vi "[ce] CalcExpress Light.vi"(5 "directives":T1={"enaNamedConst"=TRUE}, 7 "VC Handle":T5=-1, 8 "error in":errorcluster, 9 "params":T3={"autoVar"=TRUE, "enCpx"=TRUE}, 10 "repeat (1)":i32=1, 11 "expression":string) -> (0 "error out":errorcluster, 1 "value type":T4=enum."DBL Number", 3 "numeric value":dbl)   [LabVIEW 2021]
doc: "This VI evaluates CalcExpress expressions and sequential scripts. To process non-sequential scripts that contain loops and conditional branching, use <b>CSE VIs</b>. Refer to the VI help for more details.\n\n<b>VC Handle</b> specifies the handle of a variable context. CalcExpress accesses variables using this handle. Pass a valid handle to this terminal if the expression uses variables; otherwise, you can leave this input unwired.\n\n<b>expression</b> specifies the CalcExpress expression or sequential script to be executed.\n\n<b>repeat</b> control specifies the number of times an expression is evaluated. The default value is 1.\n\n<b>params</b> cluster specifies optional parameters influencing evaluation:\n <b>autoVar</b> : if it is TRUE (default) and a non-existent variable appears as the left-hand operand in the assignment operator, CalcExpress implicitly creates the variable. If it is FALSE, all variables in the expression must be explicitly created either before or during evaluation.\n <b>enCpx</b> : enables (TRUE, default) or disables (FALSE) the ability to perform operations on operands of data types other than <b>DBL Number</b>.\n\n<b>numeric value</b> returns the numeric value (<b>DBL Number</b>) of the expression.\n\n<b>value type</b> indicates the data type of the expression value.\n\n::: CalcExpress Toolkit :::\nCopyright (c) 2000-2026 Konstantin Shifershteyn. All rights reserved."
uses:
  cetypes.llb/VarMan Variable Context Handle.ctl
  cetypes.llb/CalcExpress Data Type.ctl
  cetypes.llb/CalcExpress Execution Options.ctl
  cetypes.llb/CalcExpress Instance RefNum.ctl
  cetypes.llb/CalcExpress Parsing Directives.ctl
  cersrc/celveng32.dll
panel:
  in  "CE InstanceRef Templ.":T2
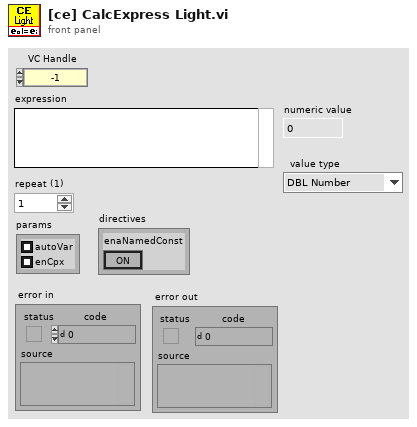
[diagram p1: front panel]
types:
  T1 = typedef "CalcExpress Parsing Directives.ctl" = cluster{"enaNamedConst":bool}
  T2 = typedef "CalcExpress Instance RefNum.ctl" = refnum<k1>
  T3 = typedef "CalcExpress Execution Options.ctl" = cluster{"autoVar":bool, "enCpx":bool}
  T4 = typedef "CalcExpress Data Type.ctl" = enum32{"String", "DBL Number", "identifier", "1D Array of DBL", "2D Array of DBL", "CDB Number", "1D Array of CDB", "2D Array of CDB", "1D Array of String", "2D Array of String", "Unknown data type"}
  T5 = typedef "VarMan Variable Context Handle.ctl" = i32
  T6 = enum32{"String", "DBL Number", "identifier", "1D Array of DBL", "2D Array of DBL", "CDB Number", "1D Array of CDB", "2D Array of CDB", "1D Array of String", "2D Array of String", "Unknown data type"}
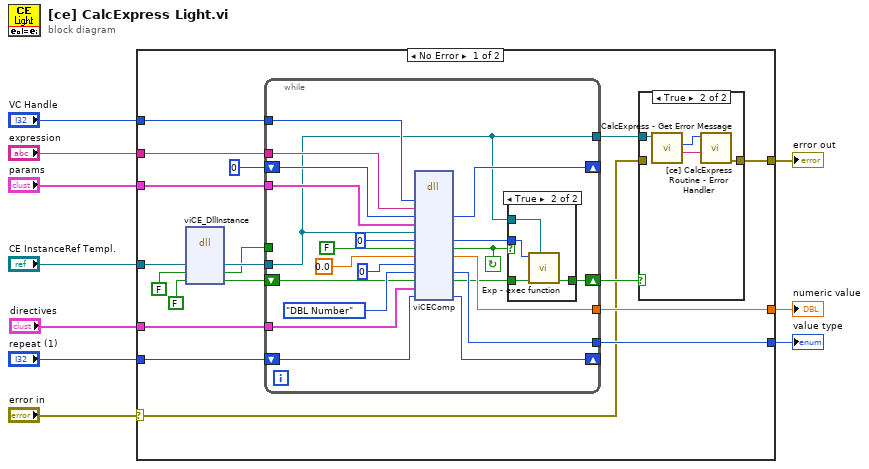
[diagram p0: block diagram]
diagram:
  n1 = case shown="No Error" "error in" {
    selector: "error in" -> [w12 w60]
    tunnel: [w23 w60] -> w10
    tunnel: [w22 _] -> w9
    tunnel: [w21 _] -> w8
    tunnel: "VC Handle" -> [w20 _]
    tunnel: "expression" -> [w19 _]
    tunnel: "params" -> [w18 _]
    tunnel: "CE InstanceRef Templ." -> [w17 _]
    tunnel: "repeat (1)" -> [w16 _]
    tunnel: "directives" -> [w11 _]
    frame No Error {
      n2 = dll-call lib="C:/LV Projects/CalcExpress 40 LV2021/vi.lib/addons/CalcExpress/cersrc/celveng*.dll" fn="viCE_DllInstance"("iRef"=w17, "newInst"=FALSE, "err_f"=FALSE) -> ("iRef"=w25:T2, "newInst"=w15:bool, "err_f"=w27:bool)  [unwired: 6 in, 2 out]
      n3 = while {
        tunnel: [w31] -> w24
        shift-left: w16 -> [w33]
        shift-right: [w32] -> _
        tunnel: [w36] -> w22
        tunnel: [w39] -> w21
        tunnel: w25 -> [w31]
        tunnel: w19 -> [w47]
        tunnel: w20 -> [w48]
        tunnel: w18 -> [w44]
        shift-left: 0 -> [w46]
        shift-right: [w45] -> _
        shift-left: w27 -> [w35]
        shift-right: [w49] -> w13
        tunnel: w15 -> [_]
        tunnel: w11 -> [w29]
        stop <- w40 continue-if-true
        n4 = dll-call lib="C:/LV Projects/CalcExpress 40 LV2021/vi.lib/addons/CalcExpress/cersrc/celveng*.dll" fn="viCEComp"("vch"=w48, "script"=w47, "idx"=w46, "cPar"=w44, "iRef"=w31, "opdNum"=0, "NE"=FALSE, "num"=0.0, "str"=u64 0, "type"=T6."DBL Number" ("data type"), "erf"=w35, "dirs"=w29, "rept"=w33) -> ("idx"=w45:i32, "opdNum"=w42:i32, "NE"=w40:bool, "num"=w39:dbl, "type"=w36:T6, "erf"=w34:bool, "rept"=w32:i32)  [unwired: 10 in, 2 out]
        n5 = case shown="True" w40 {
          tunnel: [w50 w54] -> w49
          tunnel: w34 -> [w50 w53]
          tunnel: w42 -> [_ w52]
          tunnel: w31 -> [_ w51]
          frame False {
          }
          frame True {
            n6 = call "Exp - exec function.vi"("CE InstanceRef"=w51, "error in"=w53, "ParNum"=w52) -> ("error out"=w54:bool)  [unwired: 6 in]
          }
        }
      }
      n7 = case shown="True" w13 {
        tunnel: w24 -> [_ w59]
        tunnel: [w55 w56] -> w23
        tunnel: w12 -> [w55 _]
        frame False {
        }
        frame True {
          n8 = call "CalcExpress - Get Error Message.vi"("CE InstanceRef"=w59) -> ("error description"=w58:string, "error code"=w57:i32)  [unwired: 5 in, 2 out]
          n9 = call "[ce] CalcExpress Routine - Error Handler.vi"("error msg"=w58, "error code"=w57) -> ("error out"=w56:errorcluster)  [unwired: 7 in]
        }
      }
    }
    frame Error {
    }
  }
  "error out" <- w10
  "numeric value" <- w8
  "value type" <- w9
